vi "Theta Calculation_adjust(SubVI).vi"(0 "User Input theta":dbl min=-45.0 max=45.0, 5 "Position=-85, I":dbl, 7 "Right":bool, 9 "Left":bool, 11 "User Input theta":refnum<vi>) -> (4 "Position=-85, O":dbl, 6 "Real output theta":dbl, 8 "Step diff":dbl)   [LabVIEW 2018]
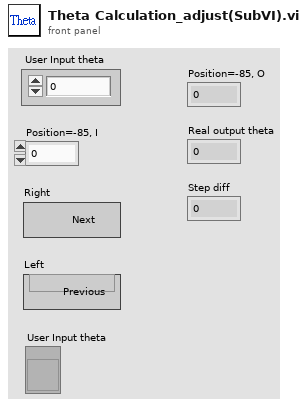
[diagram p1: front panel]
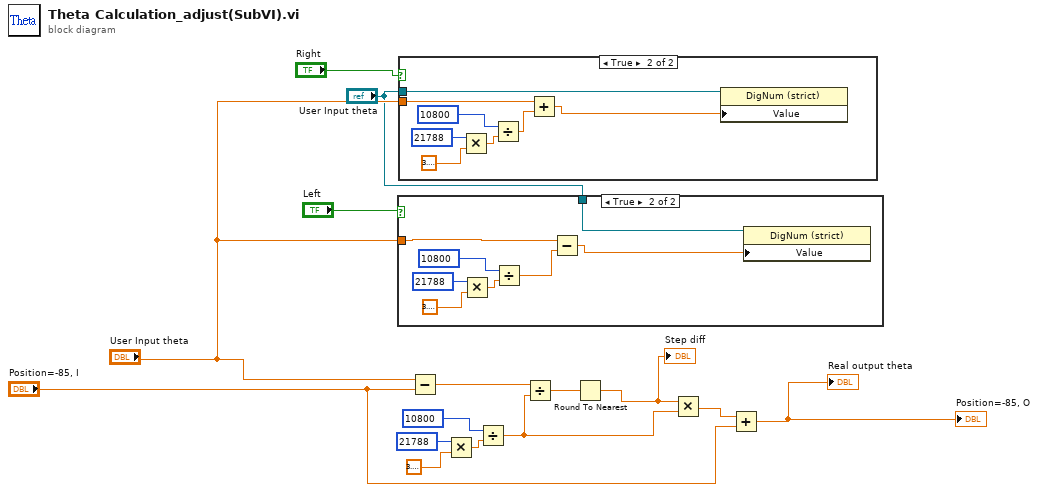
[diagram p0: block diagram]
diagram:
  n1 = case shown="True" "Left" {
    tunnel: "User Input theta" -> [_ w23]
    tunnel: "User Input theta" -> [_ w17]
    frame False {
    }
    frame True {
      n2 = Multiply(x=21788, y=3.141592653589793) -> (x*y=w21:dbl)
      n3 = Divide(x=10800, y=w21) -> (x/y=w18:dbl)
      n4 = Subtract(x=w23, y=w18) -> (x-y=w16:dbl)
      n5 = property class="DigNum (strict)"(reference=w17, "Value"=w16) -> ()  [unwired: 1 in, 2 out]
    }
  }
  n6 = case shown="True" "Right" {
    tunnel: "User Input theta" -> [_ w29]
    tunnel: "User Input theta" -> [_ w25]
    frame False {
    }
    frame True {
      n7 = Multiply(x=21788, y=3.141592653589793) -> (x*y=w28:dbl)
      n8 = Divide(x=10800, y=w28) -> (x/y=w30:dbl)
      n9 = Add(x=w29, y=w30) -> (x+y=w24:dbl)
      n10 = property class="DigNum (strict)"(reference=w25, "Value"=w24) -> ()  [unwired: 1 in, 2 out]
    }
  }
  n11 = Subtract(x="User Input theta", y="Position=-85, I") -> (x-y=w7:dbl)
  n12 = Multiply(x=21788, y=3.141592653589793) -> (x*y=w4:dbl)
  n13 = Divide(x=10800, y=w4) -> (x/y=w9:dbl)
  n14 = Divide(x=w7, y=w9) -> (x/y=w8:dbl)
  n15 = Round To Nearest(number=w8) -> (nearest integer value=w11:dbl)
  "Step diff" <- w11
  n16 = Multiply(x=w11, y=w9) -> (x*y=w2:dbl)
  n17 = Add(x=w2, y="Position=-85, I") -> (x+y=→"Real output theta" →"Position=-85, O":dbl)
